vi "Process.vi"(8 "error in":errorcluster, 11 "DAQmx":refnum<class "DAQmx.lvclass">) -> (0 "error out":errorcluster, 3 "DAQmx out":refnum<class "DAQmx.lvclass">)   [LabVIEW 2019, in "DAQmx.lvclass"]
uses:
  DAQmx.lvclass
  C:/Program Files (x86)/National Instruments/LabVIEW 2019/vi.lib/JKI/JKI SMO/SMO/SMO.lvclass
  typedefs/DAQmx.Status--enum.ctl
  typedefs/DAQmx.Commands--enum.ctl
  <vilib>/JKI/JKI SMO/SMO/SMO.lvclass/SMO.ctl
  DAQmx.lvclass/DAQmx.ctl
  typedefs/Message--Cluster.ctl
  typedefs/DAQ.Config.Timing--Cluster.ctl
  typedefs/DAQ.Config.Timing.Sampling--Cluster.ctl
  typedefs/DAQ.Config.Timing.Fs Mode--enum.ctl
  <userlib>/LevyLab/Debug/Attribute.Debug/DebugBehavior.ctl
  45607b6f-cbbd-4354-99c2-ae126d9fef0d.vi
  <vilib>/JKI/JKI SMO/SMO/Private/ReftoDVR--SMO.vi
  <vilib>/JKI/JKI SMO/SMO/SMO.lvclass
  <userlib>/LevyLab/Debug/Debug.lvlib
  <userlib>/LevyLab/Debug/Attribute.Debug/Attribute.Debug.lvclass
panel:
  out "Error":string
  out "event loop":i32
  out "acq loop":i32
  out "Command":T1
  out "Status":T2
  out "State":string
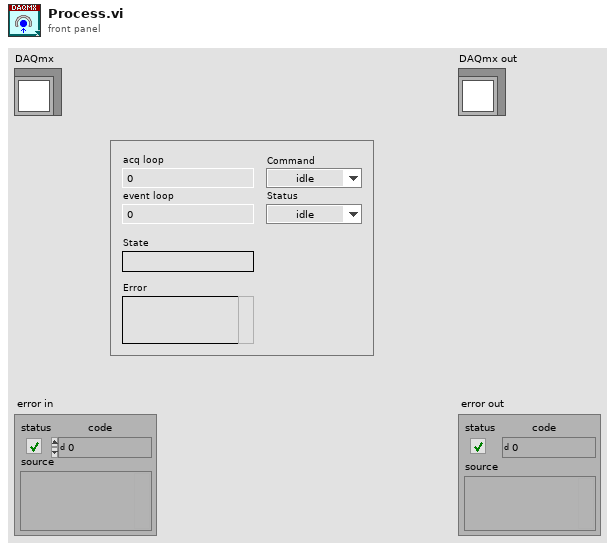
[diagram p1: front panel]
types:
  T1 = typedef "DAQmx.lvclass/DAQmx.Commands--enum.ctl" = enum16{"idle", "start", "stop", "calibrate", "auto", "exit"}
  T2 = typedef "DAQmx.lvclass/DAQmx.Status--enum.ctl" = enum16{"idle", "calibrating", "configuring", "creating", "created", "starting", "started", "stopping", "stopped", "clearing", "error"}
  T3 = typedef "Debug.lvlib/Attribute.Debug.lvclass/DebugBehavior.ctl" = enum16{"Normal", "Debug"}
  T4 = enum32{"Invalid", "Standard", "Closed", "Hidden", "Minimized", "Maximized"}
  T5 = typedef "DAQmx.lvclass/Message--Cluster.ctl" = cluster{"command":T1, "Argument":string}
  T6 = typedef "DAQmx.lvclass/DAQ.Config.Timing--Cluster.ctl" = cluster{"Sampling":T7, "sample mode":i32, "FsMode":T8, "Fs Multiplier":dbl, "Refresh Rate (Hz)":dbl, "Decimation.PreDSP":i32, "Decimation.PostDSP":i32, "Fs.Output":dbl}
  T7 = typedef "DAQmx.lvclass/DAQ.Config.Timing.Sampling--Cluster.ctl" = cluster{"Fs":dbl, "#s":i32}
  T8 = typedef "DAQmx.lvclass/DAQ.Config.Timing.Fs Mode--enum.ctl" = enum16{"Manual", "Auto Fs", "Max Fs"}
  T9 = typedef "SMO.lvclass/Protected Events.ctl" = cluster{"StopProcesses":refnum<user-event>, "AbortProcesses":refnum<user-event>, "Config Changed":refnum<user-event>, "Dependency":refnum<user-event>}
  T10 = typedef "DAQmx.lvclass/PrivateEvents--Cluster.ctl" = cluster{"Message":refnum<user-event>, "AOconfig":refnum<user-event>, "AIconfig":refnum<user-event>, "Timing":refnum<user-event>}
  T11 = cluster{"Active Device":string, "SelfCal.LastDate/Time":string, "SelfCal.LastTemp":dbl, "DevTemp":dbl, "calibration due?":bool}[]
  T12 = typedef "DAQmx.lvclass/DeviceInfo--Cluster.ctl" = cluster{"DeviceName":string, "DevIsSimulated":bool, "DeviceSerialNumber":string, "ProductType":string, "ProductCategory":i32, "ProductNumber":u32, "ChassisNumber":u32, "SlotNumber":u32, "ChassisName":string, "ChassisSerialNumber":string, "DevTemp":dbl, "SelfCal.LastDate/Time":string, "SelfCal.LastTemp":dbl, "calibration due?":bool}
  T13 = typedef "DAQmx.lvclass/DAQ.Config.AI--Cluster--Array.ctl" = T14[]
  T14 = typedef "DAQmx.lvclass/DAQ.Config.AI--Cluster.ctl" = cluster{"Channels":tag, "Coupling":T15, "Range":T16, "input terminal configuration":i32, "Type":T17}
  T15 = typedef "DAQmx.lvclass/DAQ.Config.AI.Coupling--enum.ctl" = u16
  T16 = typedef "DAQmx.lvclass/DAQ.Config.AI.Range--enum.ctl" = enum16{"±0.316", "±1.00", "±3.16", "±10.0", "±31.6", "±42.4", ""}
  T17 = typedef "DAQmx.lvclass/DAQ.Config.Device Type--enum.ctl" = enum16{"None", "USB-4431", "PXI-446x"}
  T18 = typedef "DAQmx.lvclass/DAQ.Config.AO--Cluster--Array.ctl" = T19[]
  T19 = typedef "DAQmx.lvclass/DAQ.Config.AO--Cluster.ctl" = cluster{"Channels":tag, "Range":T20, "output terminal configuration":i32, "Type":T17}
  T20 = typedef "DAQmx.lvclass/DAQ.Config.AO.Range--enum.ctl" = enum16{"±0.1", "±1.0", "±3.5", "±10.0", ""}
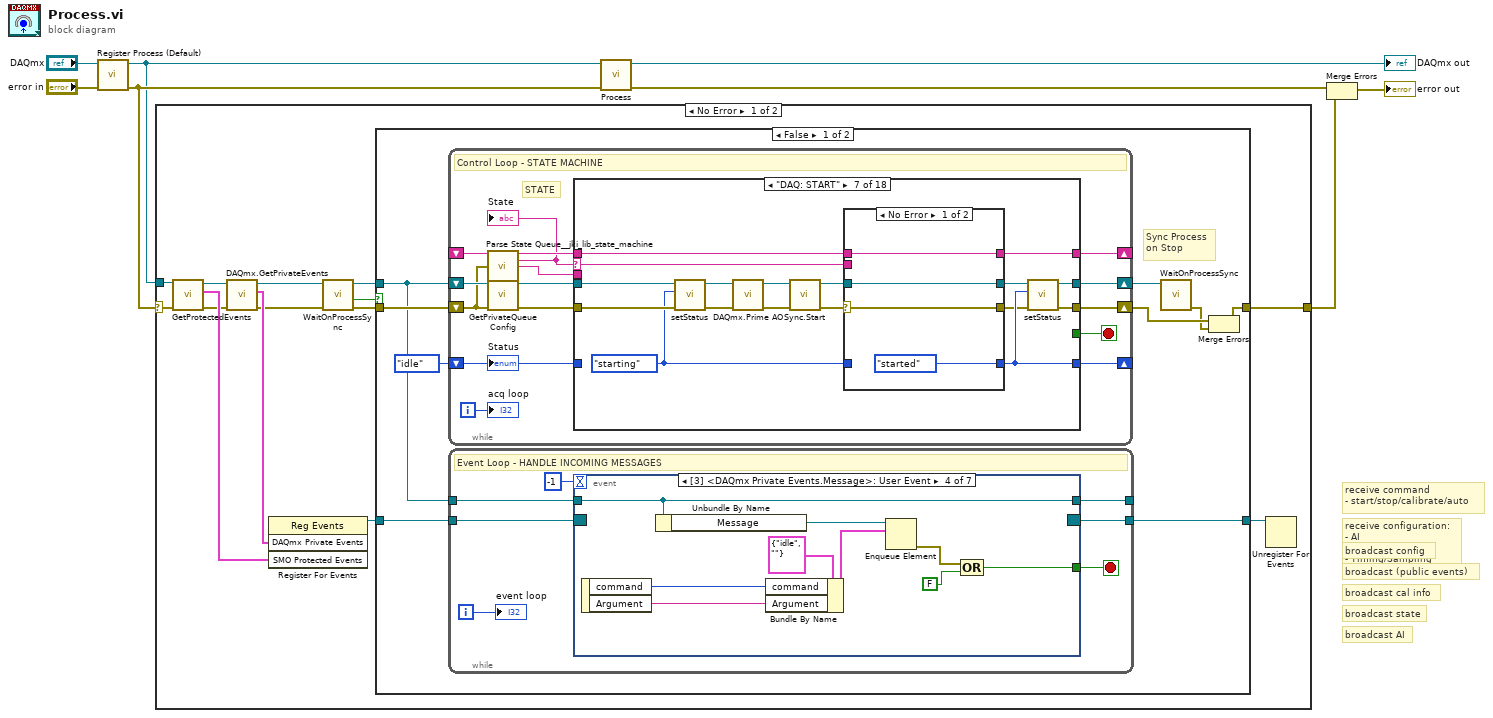
[diagram p0: block diagram]
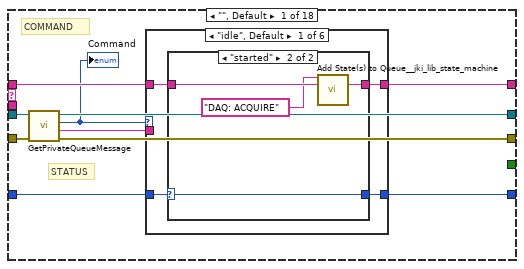
[diagram p2: hidden frame]
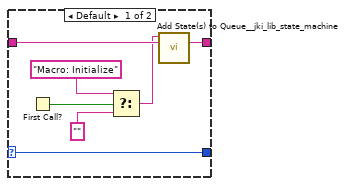
[diagram p3: hidden frame]
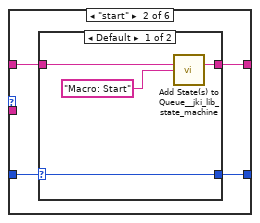
[diagram p4: hidden frame]
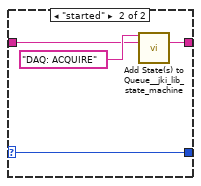
[diagram p5: hidden frame]
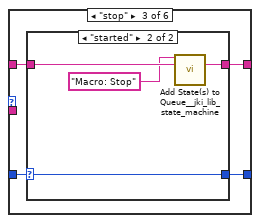
[diagram p6: hidden frame]
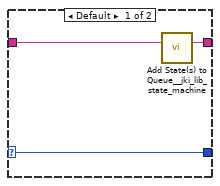
[diagram p7: hidden frame]
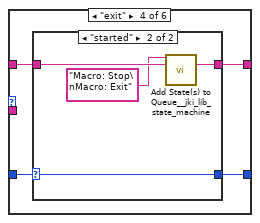
[diagram p8: hidden frame]
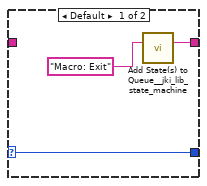
[diagram p9: hidden frame]
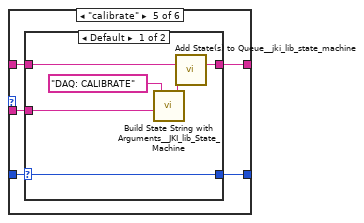
[diagram p10: hidden frame]
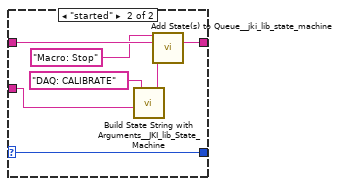
[diagram p11: hidden frame]
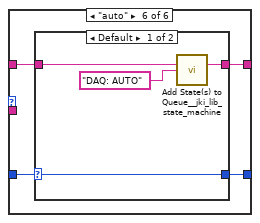
[diagram p12: hidden frame]
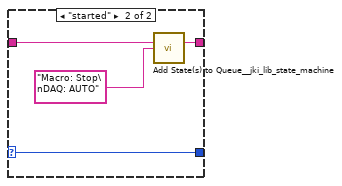
[diagram p13: hidden frame]
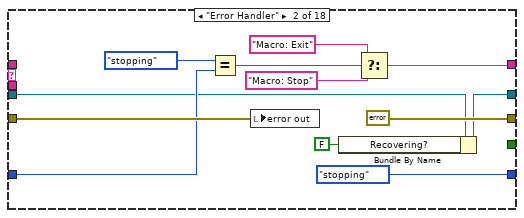
[diagram p14: hidden frame]
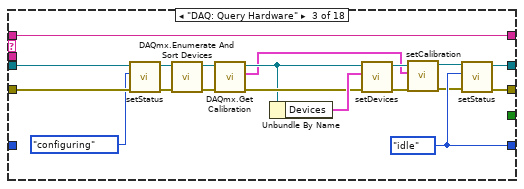
[diagram p15: hidden frame]
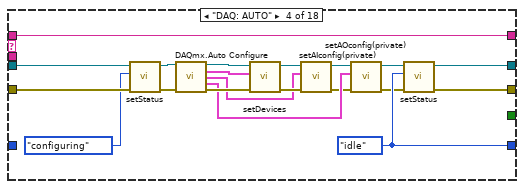
[diagram p16: hidden frame]
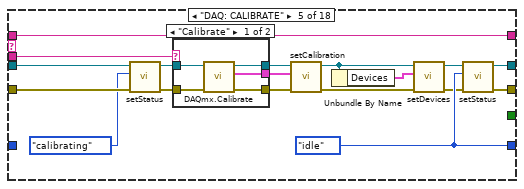
[diagram p17: hidden frame]
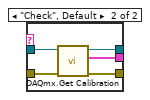
[diagram p18: hidden frame]
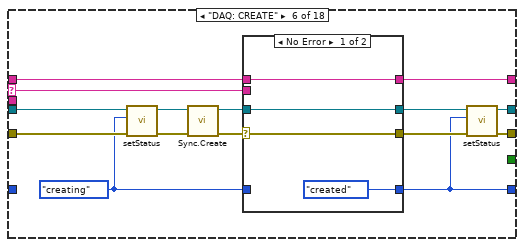
[diagram p19: hidden frame]
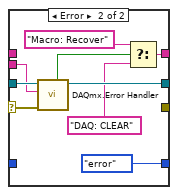
[diagram p20: hidden frame]
diagram:
  # "broadcast (public events)"
  # "receive configuration:\n- AI\n- AO\n- Timing/Sampling"
  # "receive command\n- start/stop/calibrate/auto"
  # "broadcast AI"
  # "broadcast state"
  # "broadcast cal info"
  # "broadcast config"
  n1 = call <vilib>:"Register Process (Default).vi"("error in (no error)"="error in", "SMO"="DAQmx") -> ("error out"=w3:errorcluster, "SelfRef"=w1:refnum<class "DAQmx.lvclass">)  [unwired: 8 in]
  n2 = case shown="No Error" w3 {
    selector: w3 -> [w20 w551]
    tunnel: w1 -> [w21 _]
    tunnel: [w16 w551] -> w8
    frame No Error {
      n3 = call <vilib>:"GetProtectedEvents.vi"("error in (no error)"=w20, "SMO"=w21) -> ("error out"=w13:errorcluster, "SMO Protected Events"=w22:T9, "SMO out"=w12:refnum<class "DAQmx.lvclass">)  [unwired: 7 in]
      n4 = call "DAQmx.GetPrivateEvents.vi"("error in (no error)"=w13, "DAQmx"=w12) -> ("error out"=w9:errorcluster, "DAQmx Private Events"=w11:T10, "DAQmx out"=w10:refnum<class "DAQmx.lvclass">)  [unwired: 7 in]
      n5 = register-events(w11, w22) -> (reference out=w14:refnum<event-registration>)  [unwired: 2 in, 1 out]
      n6 = call <vilib>:"WaitOnProcessSync.vi"("error in (no error)"=w9, "SMO"=w10) -> ("error out"=w18:errorcluster, "Don't run?"=w17:bool, "SMO out"=w19:refnum<class "DAQmx.lvclass">)  [unwired: 7 in]
      n7 = case shown="False" w17 {
        tunnel: w18 -> [w28 w549]
        tunnel: w19 -> [w23 _]
        tunnel: w14 -> [w30 w550]
        tunnel: [w25 w549] -> w16
        tunnel: [w29 w550] -> w15
        frame False {
          # "Sync Process\non Stop"
          n8 = while {
            shift-right: [w44] -> w31
            shift-left: w23 -> [w39]
            shift-right: [w36] -> w27
            shift-left: w28 -> [w33]
            shift-right: [w43] -> _
            shift-left: _ -> [w46]
            shift-right: [w45] -> _
            shift-left: DAQmx.Status--enum."idle" ("Status") -> [w40]
            i -> [w34]
            stop <- w32 stop-if-true
            # "STATE"
            # "Control Loop - STATE MACHINE"
            n9 = call <vilib>:"Parse State Queue__jki_lib_state_machine.vi"("State Queue"=w46, "Error In (no error)"=w33) -> ("Remaining States"=w42:string, "Current State"=w41:string, "Arguments"=w35:string)  [unwired: 11 in]
            "State" <- w41
            n10 = call "GetPrivateQueueConfig.vi"("error in (no error)"=w33, "DAQmx"=w39) -> ("error out"=w37:errorcluster, "DAQmx out"=w38:refnum<class "DAQmx.lvclass">)  [unwired: 8 in]
            n11 = case shown="\"DAQ: START\"" w41 {
              selector: w41 -> [_ _ _ _ _ w222 w249 w284 w321 w344 _ _ _ _ _ _ _ _]
              tunnel: w38 -> [w51 w137 w158 w180 w202 w228 w258 w290 w326 w349 w364 w367 w373 w387 w397 w417 w427 w491]
              tunnel: [w52 w136 w159 w175 w195 w216 w245 w281 w319 w340 w364 w367 w374 w388 w395 w411 w427 w493] -> w44
              tunnel: [w49 errorcluster {"status"=FALSE, "code"=0, "source"=""} ("error out") w160 w174 w196 w215 w244 w282 w318 w341 w363 w368 w377 w386 w394 w420 _ w492] -> w36
              tunnel: w37 -> [w50 w141 w163 w179 w201 w229 w257 w289 w327 w353 w363 w368 w377 w385 w396 w416 _ w490]
              tunnel: w35 -> [_ _ _ _ w204 _ _ _ _ _ _ _ _ _ _ _ w424 _]
              tunnel: w42 -> [w53 _ w166 w186 w194 w220 w250 w287 w322 w346 _ w370 w379 w389 w405 w419 w426 w489]
              tunnel: [w56 w139 w166 w186 w194 w221 w251 w288 w323 w345 "UI: Initialize\nDAQ: Query Hardware" ("States Out") w371 w380 w390 w406 w423 w426 w489] -> w43
              tunnel: [w54 DAQmx.Status--enum."stopping" ("Status") w161 w178 w197 w217 w248 w283 w316 w339 w362 w366 w376 w391 w404 w422 w428 w495] -> w45
              tunnel: w40 -> [w55 w140 _ _ _ _ _ w286 _ _ w362 w366 w376 w391 w404 w422 w428 w495]
              tunnel: [_ _ _ _ _ _ _ _ _ _ _ _ _ _ _ _ _ TRUE] -> w32
              frame "", Default {
                # "STATUS"
                # "COMMAND"
                n12 = call "GetPrivateQueueMessage.vi"("error in (no error)"=w50, "DAQmx"=w51) -> ("error out"=w49:errorcluster, "argument"=w47:string, "command"=w48:T1, "DAQmx out"=w52:refnum<class "DAQmx.lvclass">)  [unwired: 6 in]
                "Command" <- w48
                n13 = case shown="\"idle\", Default" w48 {
                  tunnel: w55 -> [w60 w75 w87 w98 w110 w127]
                  tunnel: [w58 w74 w86 w97 w109 w126] -> w56
                  tunnel: [w59 w73 w85 w96 w108 w125] -> w54
                  tunnel: w53 -> [w57 w72 w84 w95 w107 w124]
                  tunnel: w47 -> [_ _ _ _ w106 _]
                  frame "idle", Default {
                    n14 = case shown="\"started\"" w60 {
                      selector: w60 -> [w67 w71]
                      tunnel: [w63 w69] -> w58
                      tunnel: [w67 w71] -> w59
                      tunnel: w57 -> [w62 w70]
                      frame Default {
                        n15 = First Call?() -> (First Call?: T/F=w65:bool)
                        n16 = Select(t="Macro: Initialize" ("States Out"), s=w65, f="" ("States Out")) -> (s? t:f=w61:string)
                        n17 = call <vilib>:"Add State(s) to Queue__jki_lib_state_machine.vi"("State(s) in Front (\"\")"=w61, "State(s) in (\"\")"=w62) -> ("States Out"=w63:string)  [unwired: 13 in]
                      }
                      frame "started" {
                        n18 = call <vilib>:"Add State(s) to Queue__jki_lib_state_machine.vi"("State(s) in Front (\"\")"="DAQ: ACQUIRE" ("State(s) in (\"\")"), "State(s) in (\"\")"=w70) -> ("States Out"=w69:string)  [unwired: 13 in]
                      }
                    }
                  }
                  frame "start" {
                    n19 = case shown="Default" w75 {
                      selector: w75 -> [w79 w83]
                      tunnel: [w77 w82] -> w74
                      tunnel: [w79 w83] -> w73
                      tunnel: w72 -> [w78 w80]
                      frame Default {
                        n20 = call <vilib>:"Add State(s) to Queue__jki_lib_state_machine.vi"("State(s) in (\"\")"=w78, "State(s) at Back (\"\")"="Macro: Start" ("State(s) in (\"\")")) -> ("States Out"=w77:string)  [unwired: 13 in]
                      }
                      frame "started" {
                        n21 = call <vilib>:"Add State(s) to Queue__jki_lib_state_machine.vi"("State(s) in Front (\"\")"="DAQ: ACQUIRE" ("State(s) in (\"\")"), "State(s) in (\"\")"=w80) -> ("States Out"=w82:string)  [unwired: 13 in]
                      }
                    }
                  }
                  frame "stop" {
                    n22 = case shown="\"started\"" w87 {
                      selector: w87 -> [w90 w94]
                      tunnel: [w88 w92] -> w86
                      tunnel: [w90 w94] -> w85
                      tunnel: w84 -> [w89 w93]
                      frame Default {
                        n23 = call <vilib>:"Add State(s) to Queue__jki_lib_state_machine.vi"("State(s) in (\"\")"=w89) -> ("States Out"=w88:string)  [unwired: 14 in]
                      }
                      frame "started" {
                        n24 = call <vilib>:"Add State(s) to Queue__jki_lib_state_machine.vi"("State(s) in Front (\"\")"="Macro: Stop" ("State(s) in (\"\")"), "State(s) in (\"\")"=w93) -> ("States Out"=w92:string)  [unwired: 13 in]
                      }
                    }
                  }
                  frame "exit" {
                    n25 = case shown="\"started\"" w98 {
                      selector: w98 -> [w101 w105]
                      tunnel: [w100 w102] -> w97
                      tunnel: [w101 w105] -> w96
                      tunnel: w95 -> [_ w104]
                      frame Default {
                        n26 = call <vilib>:"Add State(s) to Queue__jki_lib_state_machine.vi"("State(s) in (\"\")"="Macro: Exit" ("State(s) in (\"\")")) -> ("States Out"=w100:string)  [unwired: 14 in]
                      }
                      frame "started" {
                        n27 = call <vilib>:"Add State(s) to Queue__jki_lib_state_machine.vi"("State(s) in Front (\"\")"="Macro: Stop\nMacro: Exit" ("State(s) in (\"\")"), "State(s) in (\"\")"=w104) -> ("States Out"=w102:string)  [unwired: 13 in]
                      }
                    }
                  }
                  frame "calibrate" {
                    n28 = case shown="Default" w110 {
                      selector: w110 -> [w116 w123]
                      tunnel: [w114 w121] -> w109
                      tunnel: [w116 w123] -> w108
                      tunnel: w107 -> [w115 w122]
                      tunnel: w106 -> [w113 w119]
                      frame Default {
                        n29 = call <vilib>:"Build State String with Arguments__JKI_lib_State_Machine.vi"("Arguments (\"\")"=w113, "State"="DAQ: CALIBRATE" ("State(s) in (\"\")")) -> ("State with Arguments"=w111:string)  [unwired: 4 in]
                        n30 = call <vilib>:"Add State(s) to Queue__jki_lib_state_machine.vi"("State(s) in (\"\")"=w115, "State(s) at Back (\"\")"=w111) -> ("States Out"=w114:string)  [unwired: 13 in]
                      }
                      frame "started" {
                        n31 = call <vilib>:"Build State String with Arguments__JKI_lib_State_Machine.vi"("Arguments (\"\")"=w119, "State"="DAQ: CALIBRATE" ("State(s) in (\"\")")) -> ("State with Arguments"=w117:string)  [unwired: 4 in]
                        n32 = call <vilib>:"Add State(s) to Queue__jki_lib_state_machine.vi"("State(s) in Front (\"\")"="Macro: Stop" ("State(s) in (\"\")"), "State(s) in (\"\")"=w122, "State(s) at Back (\"\")"=w117) -> ("States Out"=w121:string)  [unwired: 12 in]
                      }
                    }
                  }
                  frame "auto" {
                    n33 = case shown="Default" w127 {
                      selector: w127 -> [w131 w135]
                      tunnel: [w129 w133] -> w126
                      tunnel: [w131 w135] -> w125
                      tunnel: w124 -> [w130 w134]
                      frame Default {
                        n34 = call <vilib>:"Add State(s) to Queue__jki_lib_state_machine.vi"("State(s) in (\"\")"=w130, "State(s) at Back (\"\")"="DAQ: AUTO" ("State(s) in (\"\")")) -> ("States Out"=w129:string)  [unwired: 13 in]
                      }
                      frame "started" {
                        n35 = call <vilib>:"Add State(s) to Queue__jki_lib_state_machine.vi"("State(s) in (\"\")"=w134, "State(s) at Back (\"\")"="Macro: Stop\nDAQ: AUTO" ("State(s) in (\"\")")) -> ("States Out"=w133:string)  [unwired: 13 in]
                      }
                    }
                  }
                }
              }
              frame "Error Handler" {
                n36 = Equal?(x=DAQmx.Status--enum."stopping" ("Status"), y=w140) -> (x = y?=w143:bool)
                n37 = local write "error out"(w141) -> ()
                n38 = Bundle By Name(cluster=w137, "Recovering?"=FALSE ("Recovery.Recovering?")) -> (w136:refnum<class "DAQmx.lvclass">)
                n39 = Select(t="Macro: Exit", s=w143, f="Macro: Stop" ("States Out")) -> (s? t:f=w139:string)
              }
              frame "DAQ: Query Hardware" {
                w161 = DAQmx.Status--enum."idle" ("setStatus")
                n40 = call "setStatus.vi"("error in (no error)"=w163, "Status"=DAQmx.Status--enum."configuring" ("setStatus"), "DAQmx in"=w158) -> ("error out"=w164:errorcluster, "DAQmx out"=w165:refnum<class "DAQmx.lvclass">)  [unwired: 7 in]
                n41 = call "DAQmx.Enumerate And Sort Devices.vi"("error in (no error)"=w164, "DAQmx in"=w165) -> ("error out"=w157:errorcluster, "DAQmx out"=w156:refnum<class "DAQmx.lvclass">)  [unwired: 7 in, 1 out]
                n42 = call "DAQmx.Get Calibration.vi"("error in (no error)"=w157, "DAQmx in"=w156) -> ("error out"=w154:errorcluster, "Calibration out"=w148:T11, "DAQmx out"=w153:refnum<class "DAQmx.lvclass">)  [unwired: 7 in]
                n43 = Unbundle By Name(w153) -> ("Devices"=w155:T12[])
                n44 = call "setDevices.vi"("error in (no error)"=w154, "Devices"=w155, "DAQmx in"=w153) -> ("error out"=w152:errorcluster, "DAQmx out"=w151:refnum<class "DAQmx.lvclass">)  [unwired: 7 in]
                n45 = call "setCalibration.vi"("error in (no error)"=w152, "Calibration out"=w148, "DAQmx in"=w151) -> ("error out"=w149:errorcluster, "DAQmx out"=w150:refnum<class "DAQmx.lvclass">)  [unwired: 7 in]
                n46 = call "setStatus.vi"("error in (no error)"=w149, "Status"=w161, "DAQmx in"=w150) -> ("error out"=w160:errorcluster, "DAQmx out"=w159:refnum<class "DAQmx.lvclass">)  [unwired: 7 in]
              }
              frame "DAQ: AUTO" {
                w178 = DAQmx.Status--enum."idle" ("setStatus")
                n47 = call "setStatus.vi"("error in (no error)"=w179, "Status"=DAQmx.Status--enum."configuring" ("setStatus"), "DAQmx in"=w180) -> ("error out"=w182:errorcluster, "DAQmx out"=w181:refnum<class "DAQmx.lvclass">)  [unwired: 7 in]
                n48 = call "DAQmx.Auto Configure.vi"("DAQmx in"=w181, "error in (no error)"=w182) -> ("DAQmx out"=w184:refnum<class "DAQmx.lvclass">, "Devices"=w167:T12[], "Configuration.AI"=w169:T13, "Configuration.AO"=w177:T18, "error out"=w185:errorcluster)  [unwired: 9 in]
                n49 = call "setDevices.vi"("error in (no error)"=w185, "Devices"=w167, "DAQmx in"=w184) -> ("error out"=w183:errorcluster, "DAQmx out"=w176:refnum<class "DAQmx.lvclass">)  [unwired: 7 in]
                n50 = call "setAIconfig(private).vi"("error in (no error)"=w183, "AIconfig"=w169, "DAQmx in"=w176) -> ("error out"=w172:errorcluster, "DAQmx out"=w173:refnum<class "DAQmx.lvclass">)  [unwired: 7 in]
                n51 = call "setAOconfig(private).vi"("error in (no error)"=w172, "AOconfig"=w177, "DAQmx in"=w173) -> ("error out"=w170:errorcluster, "DAQmx out"=w171:refnum<class "DAQmx.lvclass">)  [unwired: 7 in]
                n52 = call "setStatus.vi"("error in (no error)"=w170, "Status"=w178, "DAQmx in"=w171) -> ("error out"=w174:errorcluster, "DAQmx out"=w175:refnum<class "DAQmx.lvclass">)  [unwired: 7 in]
              }
              frame "DAQ: CALIBRATE" {
                w197 = DAQmx.Status--enum."idle" ("Status")
                n53 = call "setStatus.vi"("error in (no error)"=w201, "Status"=DAQmx.Status--enum."calibrating" ("setStatus"), "DAQmx in"=w202) -> ("error out"=w199:errorcluster, "DAQmx out"=w198:refnum<class "DAQmx.lvclass">)  [unwired: 7 in]
                n54 = case shown="\"Calibrate\"" w204 {
                  tunnel: w198 -> [w209 w214]
                  tunnel: [w208 w213] -> w188
                  tunnel: [w206 w212] -> w203
                  tunnel: w199 -> [w207 w211]
                  tunnel: [w205 w210] -> w193
                  frame "Calibrate" {
                    n55 = call "DAQmx.Calibrate.vi"("error in (no error)"=w207, "DAQmx in"=w209) -> ("error out"=w206:errorcluster, "Calibration out"=w205:T11, "DAQmx out"=w208:refnum<class "DAQmx.lvclass">)  [unwired: 7 in]
                  }
                  frame "Check", Default {
                    n56 = call "DAQmx.Get Calibration.vi"("error in (no error)"=w211, "DAQmx in"=w214) -> ("error out"=w212:errorcluster, "Calibration out"=w210:T11, "DAQmx out"=w213:refnum<class "DAQmx.lvclass">)  [unwired: 7 in]
                  }
                }
                n57 = call "setCalibration.vi"("error in (no error)"=w203, "Calibration out"=w193, "DAQmx in"=w188) -> ("error out"=w191:errorcluster, "DAQmx out"=w187:refnum<class "DAQmx.lvclass">)  [unwired: 7 in]
                n58 = Unbundle By Name(w187) -> ("Devices"=w192:T12[])
                n59 = call "setDevices.vi"("error in (no error)"=w191, "Devices"=w192, "DAQmx in"=w187) -> ("error out"=w189:errorcluster, "DAQmx out"=w190:refnum<class "DAQmx.lvclass">)  [unwired: 7 in]
                n60 = call "setStatus.vi"("error in (no error)"=w189, "Status"=w197, "DAQmx in"=w190) -> ("error out"=w196:errorcluster, "DAQmx out"=w195:refnum<class "DAQmx.lvclass">)  [unwired: 7 in]
              }
              frame "DAQ: CREATE" {
                w223 = DAQmx.Status--enum."creating" ("Status")
                n61 = call "setStatus.vi"("error in (no error)"=w229, "Status"=w223, "DAQmx in"=w228) -> ("error out"=w226:errorcluster, "DAQmx out"=w227:refnum<class "DAQmx.lvclass">)  [unwired: 7 in]
                n62 = call "Sync.Create.vi"("error in"=w226, "DAQmx in"=w227) -> ("error out"=w224:errorcluster, "DAQmx out"=w225:refnum<class "DAQmx.lvclass">)  [unwired: 8 in]
                n63 = case shown="No Error" w224 {
                  selector: w224 -> [w230 w241]
                  tunnel: w225 -> [w231 w242]
                  tunnel: [w230 _] -> w218
                  tunnel: [w231 w239] -> w219
                  tunnel: [DAQmx.Status--enum."created" ("Status") DAQmx.Status--enum."error" ("Status")] -> w217
                  tunnel: w223 -> [_ _]
                  tunnel: w222 -> [_ w238]
                  tunnel: [w233 w234] -> w221
                  tunnel: w220 -> [w233 _]
                  frame No Error {
                  }
                  frame Error {
                    n64 = call "DAQmx.Error Handler.vi"("error in (no error)"=w241, "[error source] (\" \")"=w238, "DAQmx in"=w242) -> ("DAQmx out"=w239:refnum<class "DAQmx.lvclass">, "retry?"=w237:bool)  [unwired: 4 in, 3 out]
                    n65 = Select(t="Macro: Recover", s=w237, f="DAQ: CLEAR" ("t")) -> (s? t:f=w234:string)
                  }
                }
                n66 = call "setStatus.vi"("error in (no error)"=w218, "Status"=w217, "DAQmx in"=w219) -> ("error out"=w215:errorcluster, "DAQmx out"=w216:refnum<class "DAQmx.lvclass">)  [unwired: 7 in]
              }
              frame "DAQ: START" {
                w252 = DAQmx.Status--enum."starting" ("Status")
                n67 = call "setStatus.vi"("error in (no error)"=w257, "Status"=w252, "DAQmx in"=w258) -> ("error out"=w256:errorcluster, "DAQmx out"=w254:refnum<class "DAQmx.lvclass">)  [unwired: 7 in]
                n68 = call "DAQmx.Prime AO.vi"("error in (no error)"=w256, "DAQmx in"=w254) -> ("error out"=w255:errorcluster, "DAQmx out"=w243:refnum<class "DAQmx.lvclass">)  [unwired: 8 in]
                n69 = call "Sync.Start.vi"("error in"=w255, "DAQmx in"=w243) -> ("error out"=w253:errorcluster, "DAQmx out"=w259:refnum<class "DAQmx.lvclass">)  [unwired: 8 in]
                n70 = case shown="No Error" w253 {
                  selector: w253 -> [w260 w270]
                  tunnel: w259 -> [w261 w271]
                  tunnel: [w260 _] -> w246
                  tunnel: [w261 w269] -> w247
                  tunnel: [DAQmx.Status--enum."started" ("Status") DAQmx.Status--enum."error" ("Status")] -> w248
                  tunnel: w252 -> [_ _]
                  tunnel: [w263 w267] -> w251
                  tunnel: w250 -> [w263 _]
                  tunnel: w249 -> [_ w272]
                  frame No Error {
                  }
                  frame Error {
                    n71 = call "DAQmx.Error Handler.vi"("error in (no error)"=w270, "[error source] (\" \")"=w272, "DAQmx in"=w271) -> ("DAQmx out"=w269:refnum<class "DAQmx.lvclass">, "retry?"=w266:bool)  [unwired: 4 in, 3 out]
                    n72 = Select(t="Macro: Recover", s=w266, f="DAQ: CLEAR" ("t")) -> (s? t:f=w267:string)
                  }
                }
                n73 = call "setStatus.vi"("error in (no error)"=w246, "Status"=w248, "DAQmx in"=w247) -> ("error out"=w244:errorcluster, "DAQmx out"=w245:refnum<class "DAQmx.lvclass">)  [unwired: 7 in]
              }
              frame "DAQ: ACQUIRE" {
                n74 = call "getWFMQueue.vi"("error in (no error)"=w289, "wait for min buffer?"=FALSE, "DAQmx in"=w290) -> ("error out"=w279:errorcluster, "DAQmx out"=w280:refnum<class "DAQmx.lvclass">)  [unwired: 6 in, 1 out]
                n75 = call "Sync.Acquire.vi"("error in (no error)"=w279, "DAQmx in"=w280) -> ("error out"=w278:errorcluster, "DAQmx out"=w277:refnum<class "DAQmx.lvclass">)  [unwired: 8 in]
                n76 = call "setWaveforms.vi"("error in (no error)"=w278, "DAQmx in"=w277) -> ("error out"=w275:errorcluster, "DAQmx out"=w276:refnum<class "DAQmx.lvclass">)  [unwired: 8 in]
                n77 = call "Scope.vi"("error in (no error)"=w275, "DAQmx in"=w276) -> ("error out"=w274:errorcluster, "DAQmx out"=w273:refnum<class "DAQmx.lvclass">)  [unwired: 8 in]
                n78 = case shown="No Error" w274 {
                  selector: w274 -> [_ w306]
                  tunnel: [w298 w311] -> w288
                  tunnel: w273 -> [w295 w315]
                  tunnel: [w293 w313] -> w281
                  tunnel: w287 -> [w298 _]
                  tunnel: w286 -> [w297 _]
                  tunnel: w284 -> [_ w308]
                  tunnel: [w297 w309] -> w283
                  tunnel: [w292 w314] -> w282
                  frame No Error {
                    n79 = call "Is Value Changed.vim"("value"=w297) -> ("changed or first call?"=w296:bool)
                    n80 = case shown="True" w296 {
                      tunnel: w295 -> [w299 w303]
                      tunnel: [w299 w302] -> w294
                      tunnel: [_ w301] -> w291
                      tunnel: w297 -> [_ w300]
                      frame False {
                      }
                      frame True {
                        n81 = call "setStatus.vi"("Status"=w300, "DAQmx in"=w303) -> ("error out"=w301:errorcluster, "DAQmx out"=w302:refnum<class "DAQmx.lvclass">)  [unwired: 8 in]
                      }
                    }
                    n82 = call "DAQmx.Acquire Recovery.vi"("error in (no error)"=w291, "DAQmx in"=w294) -> ("error out"=w292:errorcluster, "DAQmx out"=w293:refnum<class "DAQmx.lvclass">)  [unwired: 8 in]
                  }
                  frame Error {
                    w309 = DAQmx.Status--enum."error" ("t")
                    n83 = call "DAQmx.Error Handler.vi"("error in (no error)"=w306, "[error source] (\" \")"=w308, "DAQmx in"=w315) -> ("[error Description] (\" \")"=→"Error":string, "DAQmx out"=w305:refnum<class "DAQmx.lvclass">, "retry?"=w304:bool)  [unwired: 4 in, 2 out]
                    n84 = Select(t="Macro: Recover", s=w304, f="Macro: Stop" ("t")) -> (s? t:f=w311:string)
                    n85 = call "setStatus.vi"("Status"=w309, "DAQmx in"=w305) -> ("error out"=w314:errorcluster, "DAQmx out"=w313:refnum<class "DAQmx.lvclass">)  [unwired: 8 in]
                  }
                }
              }
              frame "DAQ: STOP" {
                w316 = DAQmx.Status--enum."stopped" ("Status")
                n86 = call "setStatus.vi"("error in (no error)"=w327, "Status"=DAQmx.Status--enum."stopping", "DAQmx in"=w326) -> ("error out"=w329:errorcluster, "DAQmx out"=w330:refnum<class "DAQmx.lvclass">)  [unwired: 7 in]
                n87 = call "Sync.Stop.vi"("error in (no error)"=w329, "DAQmx in"=w330) -> ("error out"=w325:errorcluster, "DAQmx out"=w328:refnum<class "DAQmx.lvclass">)  [unwired: 8 in]
                n88 = case shown="No Error" w325 {
                  selector: w325 -> [w331 w337]
                  tunnel: w328 -> [w333 w335]
                  tunnel: [w333 w336] -> w320
                  tunnel: [w332 w334] -> w323
                  tunnel: w322 -> [w332 w334]
                  tunnel: w321 -> [_ w338]
                  tunnel: [w331 _] -> w317
                  frame No Error {
                  }
                  frame Error {
                    n89 = call "DAQmx.Error Handler.vi"("error in (no error)"=w337, "[error source] (\" \")"=w338, "DAQmx in"=w335) -> ("DAQmx out"=w336:refnum<class "DAQmx.lvclass">)  [unwired: 4 in, 4 out]
                  }
                }
                n90 = call "setStatus.vi"("error in (no error)"=w317, "Status"=w316, "DAQmx in"=w320) -> ("error out"=w318:errorcluster, "DAQmx out"=w319:refnum<class "DAQmx.lvclass">)  [unwired: 7 in]
              }
              frame "DAQ: CLEAR" {
                w339 = DAQmx.Status--enum."idle" ("Status")
                n91 = call "setStatus.vi"("error in (no error)"=w353, "Status"=DAQmx.Status--enum."clearing", "DAQmx in"=w349) -> ("error out"=w351:errorcluster, "DAQmx out"=w352:refnum<class "DAQmx.lvclass">)  [unwired: 7 in]
                n92 = call "Sync.Destroy.vi"("error in (no error)"=w351, "DAQmx in"=w352) -> ("error out"=w347:errorcluster, "DAQmx out"=w350:refnum<class "DAQmx.lvclass">)  [unwired: 8 in]
                n93 = case shown="No Error" w347 {
                  selector: w347 -> [w355 w359]
                  tunnel: w350 -> [w356 w360]
                  tunnel: [w356 w358] -> w343
                  tunnel: [w355 _] -> w342
                  tunnel: w346 -> [w354 w357]
                  tunnel: [w354 w357] -> w345
                  tunnel: w344 -> [_ w361]
                  frame No Error {
                  }
                  frame Error {
                    n94 = call "DAQmx.Error Handler.vi"("error in (no error)"=w359, "[error source] (\" \")"=w361, "DAQmx in"=w360) -> ("DAQmx out"=w358:refnum<class "DAQmx.lvclass">)  [unwired: 4 in, 4 out]
                  }
                }
                n95 = call "setStatus.vi"("error in (no error)"=w342, "Status"=w339, "DAQmx in"=w343) -> ("error out"=w341:errorcluster, "DAQmx out"=w340:refnum<class "DAQmx.lvclass">)  [unwired: 7 in]
              }
              frame "Macro: Initialize" {
              }
              frame "Macro: Start" {
                n96 = call <vilib>:"Add State(s) to Queue__jki_lib_state_machine.vi"("State(s) in Front (\"\")"="DAQ: CREATE\nDAQ: START\nDAQ: ACQUIRE" ("State(s) in Front (\"\")"), "State(s) in (\"\")"=w370) -> ("States Out"=w371:string)  [unwired: 13 in]
              }
              frame "Macro: Stop" {
                w372 = waveform(dbl)[] [] ("Recovery.Pending AO")
                n97 = Bundle By Name(cluster=w373, "Recovering?"=FALSE ("Recovery.Recovering?"), "Pending AO"=w372, "Pending REF_X"=w372, "Pending REF_Y"=w372) -> (w374:refnum<class "DAQmx.lvclass">)
                n98 = call <vilib>:"Add State(s) to Queue__jki_lib_state_machine.vi"("State(s) in Front (\"\")"="DAQ: STOP\nDAQ: CLEAR" ("State(s) in Front (\"\")"), "State(s) in (\"\")"=w379) -> ("States Out"=w380:string)  [unwired: 13 in]
              }
              frame "Macro: Recover" {
                n99 = call "DAQmx.Recovery Error Handler.vi"("error in (no error)"=w385, "DAQmx in"=w387) -> ("error out"=w386:errorcluster, "retry?"=w384:bool, "DAQmxout"=w388:refnum<class "DAQmx.lvclass">)  [unwired: 7 in]
                n100 = Select(t="DAQ: STOP\nDAQ: CLEAR\nDAQ: CREATE\nDAQ: START\nDAQ: ACQUIRE" ("State(s) in Front (\"\")"), s=w384, f="Macro: Stop" ("State(s) in Front (\"\")")) -> (s? t:f=w382:string)
                n101 = call <vilib>:"Add State(s) to Queue__jki_lib_state_machine.vi"("State(s) in Front (\"\")"=w382, "State(s) in (\"\")"=w389) -> ("States Out"=w390:string)  [unwired: 13 in]
              }
              frame "Macro: Exit" {
                n102 = call <userlib>:"Get Debug Mode.vi"("error in (no error)"=w396, "SMO"=w397) -> ("error out"=w394:errorcluster, "Behavior"=w400:T3, "SMO out"=w395:refnum<class "DAQmx.lvclass">)  [unwired: 7 in]
                n103 = Equal?(x=DebugBehavior."Debug", y=w400) -> (x = y?=w403:bool)
                n104 = Select(t="Open", s=w403, f="Close") -> (s? t:f=w401:string)
                n105 = Format Into String(format string="UI: Front Panel State >> %s\nexit" ("State(s) in Front (\"\")"), w401) -> (resulting string=w392:string)  [unwired: 2 in, 1 out]
                n106 = call <vilib>:"Add State(s) to Queue__jki_lib_state_machine.vi"("State(s) in Front (\"\")"=w392, "State(s) in (\"\")"=w405) -> ("States Out"=w406:string)  [unwired: 13 in]
              }
              frame "UI: Initialize" {
                n107 = call <userlib>:"Get Debug Mode.vi"("error in (no error)"=w416, "SMO"=w417) -> ("error out"=w410:errorcluster, "Behavior"=w409:T3, "SMO out"=w411:refnum<class "DAQmx.lvclass">)  [unwired: 7 in]
                n108 = Equal?(x=DebugBehavior."Debug", y=w409) -> (x = y?=w418:bool)
                n109 = Select(t="Open", s=w418, f="Close") -> (s? t:f=w414:string)
                n110 = Format Into String(format string="UI: Front Panel State >> %s" ("State(s) in Front (\"\")"), w414) -> (resulting string=w412:string)  [unwired: 2 in, 1 out]
                n111 = call <userlib>:"Fit VI window to Largest Dec__ogtk.vi"("error in (no error)"=w410, "border spacing (2 px)"=0) -> ("error out"=w420:errorcluster)  [unwired: 4 in, 1 out]
                n112 = call <vilib>:"Add State(s) to Queue__jki_lib_state_machine.vi"("State(s) in Front (\"\")"=w412, "State(s) in (\"\")"=w419) -> ("States Out"=w423:string)  [unwired: 13 in]
              }
              frame "UI: Front Panel State" {
                n113 = control-ref of="Current VI Reference"() -> (w425:refnum<vi>)
                n114 = case shown="\"Minimize\", \"Minimized\"" w424 {
                  tunnel: [w435 w448 w459 w471 w483] -> _
                  tunnel: w425 -> [w434 w446 w458 w470 w482]
                  frame "Open", "Standard", Default {
                    w429 = T4."Standard" ("State")
                    n115 = property class="VI"(reference=w434) -> (reference out=w432:refnum<vi>, error out=w433:errorcluster, "FP.State"=w431:T4)  [unwired: 1 in]
                    n116 = Not Equal?(x=w431, y=w429) -> (x != y?=w430:bool)
                    n117 = case shown="True" w430 {
                      tunnel: [w439 w441] -> w435
                      tunnel: w433 -> [w438 w441]
                      tunnel: w432 -> [w437 _]
                      tunnel: w429 -> [w436 _]
                      frame True {
                        n118 = invoke class="VI" method="FP.Open"(reference=w437, error in=w438, "Activate"=TRUE, "State"=w436) -> (error out=w439:errorcluster)  [unwired: 1 in, 4 out]
                      }
                      frame False {
                      }
                    }
                  }
                  frame "Close", "Closed" {
                    n119 = property class="VI"(reference=w446) -> (reference out=w445:refnum<vi>, error out=w447:errorcluster, "FP.State"=w443:T4)  [unwired: 1 in]
                    n120 = Not Equal?(x=w443, y=T4."Closed" ("Front Panel Window:State")) -> (x != y?=w442:bool)
                    n121 = case shown="True" w442 {
                      tunnel: [w449 w452] -> w448
                      tunnel: w447 -> [w449 w451]
                      tunnel: w445 -> [_ w450]
                      frame False {
                      }
                      frame True {
                        n122 = invoke class="VI" method="FP.Close"(reference=w450, error in=w451) -> (error out=w452:errorcluster)  [unwired: 1 in, 2 out]
                      }
                    }
                  }
                  frame "Hidden", "Hide" {
                    w453 = T4."Hidden" ("State")
                    n123 = property class="VI"(reference=w458) -> (reference out=w456:refnum<vi>, error out=w457:errorcluster, "FP.State"=w455:T4)  [unwired: 1 in]
                    n124 = Not Equal?(x=w455, y=w453) -> (x != y?=w454:bool)
                    n125 = case shown="True" w454 {
                      tunnel: [w463 w464] -> w459
                      tunnel: w457 -> [w462 w464]
                      tunnel: w456 -> [w461 _]
                      tunnel: w453 -> [w460 _]
                      frame True {
                        n126 = invoke class="VI" method="FP.Open"(reference=w461, error in=w462, "State"=w460) -> (error out=w463:errorcluster)  [unwired: 2 in, 4 out]
                      }
                      frame False {
                      }
                    }
                  }
                  frame "Minimize", "Minimized" {
                    w465 = T4."Minimized" ("State")
                    n127 = property class="VI"(reference=w470) -> (reference out=w468:refnum<vi>, error out=w469:errorcluster, "FP.State"=w467:T4)  [unwired: 1 in]
                    n128 = Not Equal?(x=w467, y=w465) -> (x != y?=w466:bool)
                    n129 = case shown="True" w466 {
                      tunnel: [w475 w476] -> w471
                      tunnel: w469 -> [w474 w476]
                      tunnel: w468 -> [w473 _]
                      tunnel: w465 -> [w472 _]
                      frame True {
                        n130 = invoke class="VI" method="FP.Open"(reference=w473, error in=w474, "State"=w472) -> (error out=w475:errorcluster)  [unwired: 2 in, 4 out]
                      }
                      frame False {
                      }
                    }
                  }
                  frame "Maximize", "Maximized" {
                    w477 = T4."Maximized" ("State")
                    n131 = property class="VI"(reference=w482) -> (reference out=w480:refnum<vi>, error out=w481:errorcluster, "FP.State"=w479:T4)  [unwired: 1 in]
                    n132 = Not Equal?(x=w479, y=w477) -> (x != y?=w478:bool)
                    n133 = case shown="True" w478 {
                      tunnel: [w487 w488] -> w483
                      tunnel: w481 -> [w486 w488]
                      tunnel: w480 -> [w485 _]
                      tunnel: w477 -> [w484 _]
                      frame True {
                        n134 = invoke class="VI" method="FP.Open"(reference=w485, error in=w486, "State"=w484) -> (error out=w487:errorcluster)  [unwired: 2 in, 4 out]
                      }
                      frame False {
                      }
                    }
                  }
                }
              }
              frame "exit" {
                n135 = call <vilib>:"SelfTerminate.vi"("error in (no error)"=w490, "SMO in"=w491) -> ("error out"=w492:errorcluster, "SMO out"=w493:refnum<class "DAQmx.lvclass">)  [unwired: 8 in]
              }
            }
            "Status" <- w40
            "acq loop" <- w34
          }
          n136 = while {
            tunnel: w30 -> [w501]
            tunnel: [w500] -> w29
            tunnel: [w498] -> _
            tunnel: w23 -> [w497]
            i -> [w496]
            stop <- w499 stop-if-true
            # "Event Loop - HANDLE INCOMING MESSAGES"
            n137 = event shown="[3] <DAQmx Private Events.Message>: User Event" {
              selector: w501 -> [_ _ _ _ _ _ _]
              dyn-events: [_ _ _ _ _ _ _] -> w500
              timeout: -1 -> [_ _ _ _ _ _ _]
              tunnel: [_ TRUE TRUE w527 w534 w540 w548] -> w499
              tunnel: [w503 w510 w516 w525 w531 w538 w545] -> w498
              tunnel: w497 -> [w503 w510 w516 w525 w531 w538 w545]
              event Timeout {
                n138 = event-data() -> ()  [unwired: 1 in, 1 out]
              }
              event User Event {
                # "Stop SMO"
                n139 = event-data() -> ()  [unwired: 1 in, 1 out]
                n140 = Unbundle By Name(w510) -> ("Message"=w507:refnum<queue>)
                n141 = Bundle By Name(cluster=T5 {"command"=enum."idle", "Argument"=""} ("Message"), "command"=DAQmx.Commands--enum."exit" ("notification")) -> (w506:T5)
                n142 = Enqueue Element(queue=w507, element=w506) -> (error out=w508:errorcluster)  [unwired: 2 in, 2 out]
                n143 = Compound Arithmetic op=OR(w508, FALSE) -> ()  [unwired: 1 out]
              }
              event User Event {
                # "Abort SMO"
                n144 = event-data() -> ()  [unwired: 1 in, 1 out]
                n145 = Unbundle By Name(w516) -> ("Message"=w515:refnum<queue>)
                n146 = Bundle By Name(cluster=T5 {"command"=enum."idle", "Argument"=""} ("Message"), "command"=DAQmx.Commands--enum."exit" ("notification")) -> (w512:T5)
                n147 = Enqueue Element(queue=w515, element=w512) -> (error out=w517:errorcluster)  [unwired: 2 in, 2 out]
                n148 = Compound Arithmetic op=OR(w517, FALSE) -> ()  [unwired: 1 out]
              }
              event User Event {
                n149 = event-data() -> ("command"=w523:T1, "Argument"=w522:string)  [unwired: 1 in]
                n150 = Unbundle By Name(w525) -> ("Message"=w520:refnum<queue>)
                n151 = Bundle By Name(cluster=T5 {"command"=enum."idle", "Argument"=""} ("Message"), "command"=w523, "Argument"=w522) -> (w521:T5)
                n152 = Enqueue Element(queue=w520, element=w521) -> (error out=w526:errorcluster)  [unwired: 2 in, 2 out]
                n153 = Compound Arithmetic op=OR(w526, FALSE) -> (w527:bool)
              }
              event User Event {
                n154 = event-data() -> ("AOconfig"=w529:T18)  [unwired: 1 in]
                n155 = Unbundle By Name(w531) -> ("AOconfig"=w530:refnum<queue>)
                n156 = Enqueue Element(queue=w530, element=w529) -> (error out=w532:errorcluster)  [unwired: 2 in, 2 out]
                n157 = Compound Arithmetic op=OR(w532, FALSE) -> (w534:bool)
              }
              event User Event {
                n158 = event-data() -> ("AIconfig"=w536:T13)  [unwired: 1 in]
                n159 = Unbundle By Name(w538) -> ("AIconfig"=w535:refnum<queue>)
                n160 = Enqueue Element(queue=w535, element=w536) -> (error out=w537:errorcluster)  [unwired: 2 in, 2 out]
                n161 = Compound Arithmetic op=OR(w537, FALSE) -> (w540:bool)
              }
              event User Event {
                n162 = event-data() -> ("Sampling"=w544:T7)  [unwired: 1 in]
                n163 = Unbundle By Name(w545) -> ("Timing"=w542:refnum<queue>)
                n164 = Bundle By Name(cluster=T6 {"Sampling"={"Fs"=1000.0, "#s"=128}, "sample mode"=10123, "FsMode"=enum."Manual", "Fs Multiplier"=1.0, "Refresh Rate (Hz)"=10.0, "Decimation.PreDSP"=1, "Decimation.PostDSP"=1, "Fs.Output"=204789.0} ("Timing"), "Sampling"=w544) -> (w541:T6)
                n165 = Enqueue Element(queue=w542, element=w541) -> (error out=w543:errorcluster)  [unwired: 2 in, 2 out]
                n166 = Compound Arithmetic op=OR(w543, FALSE) -> (w548:bool)
              }
            }
            "event loop" <- w496
          }
          n167 = call <vilib>:"WaitOnProcessSync.vi"("SMO"=w31) -> ("error out"=w26:errorcluster)  [unwired: 8 in, 2 out]
          n168 = Merge Errors(w27, w26) -> (w25:errorcluster)
        }
        frame True {
        }
      }
      n169 = Unregister For Events(event registration refnum=w15) -> ()  [unwired: 1 in, 1 out]
    }
    frame Error {
    }
  }
  n170 = call-parent "Process.vi"("error in"=w3, "SMO"=w1) -> ("error out"=w7:errorcluster, "SMO out"=→"DAQmx out":refnum<class "DAQmx.lvclass">)  [unwired: 8 in]
  n171 = Merge Errors(w7, w8) -> (→"error out":errorcluster)
